vi "Get Largest Decoration Reference.vi"(8 "error in (no error)":errorcluster, 10 "VI reference (calling)":refnum<vi>, 11 "Dialog in":refnum<class "Dialog.lvclass">) -> (0 "error out":errorcluster, 2 "VI reference (dup)":refnum<vi>, 3 "Dialog out":refnum<class "Dialog.lvclass">)   [LabVIEW 2012, in "Dialog.lvlib" / "Dialog.lvclass"]
uses:
  Dialog.lvclass
  Dialog.lvclass/Dialog.ctl
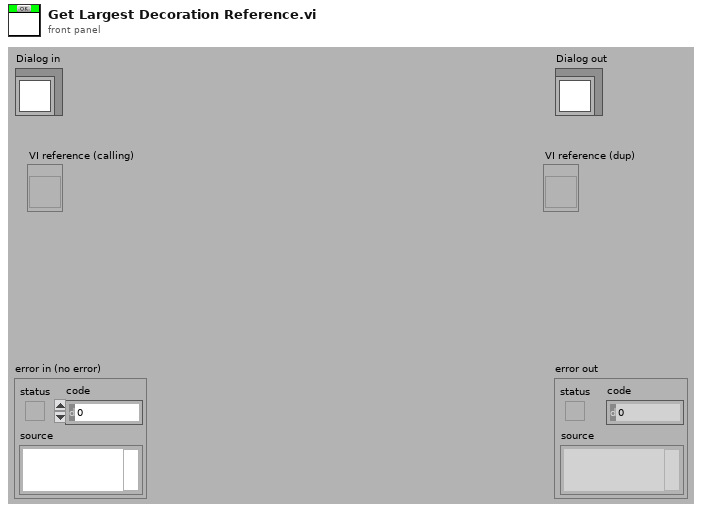
[diagram p1: front panel]
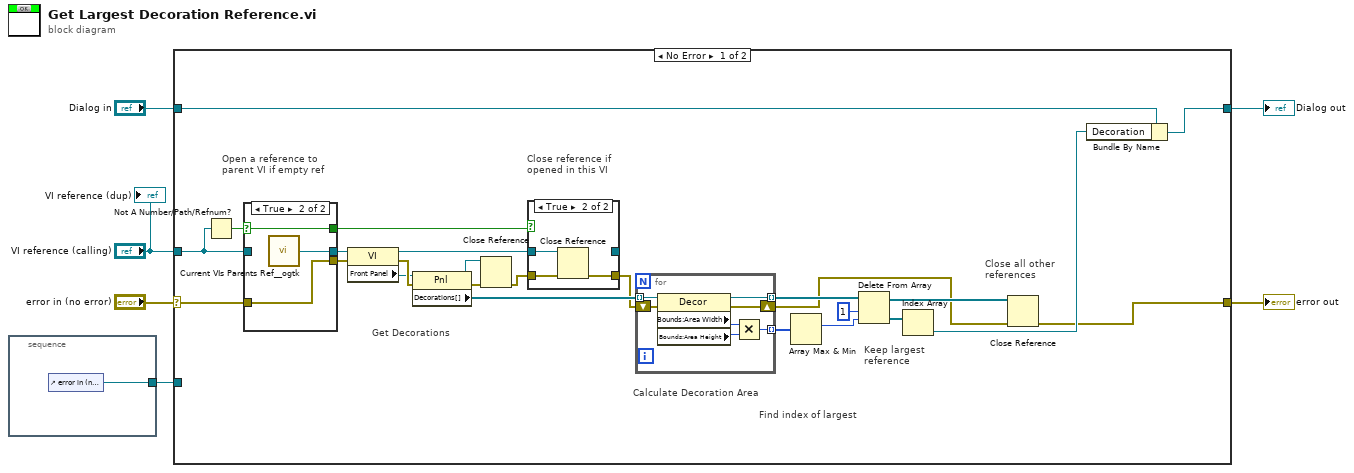
[diagram p0: block diagram]
diagram:
  n1 = stacked-sequence {
    tunnel: [w7] -> w1
    frame #0 {
      n2 = control-ref of="error in (no error)"() -> (w7:refnum<vi>)
    }
  }
  n3 = case shown="No Error" "error in (no error)" {
    selector: "error in (no error)" -> [w25 w52]
    tunnel: [w8 w52] -> w5
    tunnel: [w29 w51] -> w3
    tunnel: "Dialog in" -> [w30 w51]
    tunnel: "VI reference (calling)" -> [w26 _]
    tunnel: w1 -> [_ _]
    frame No Error {
      # "Close all other\nreferences"
      # "Keep largest\nreference"
      # "Find index of largest"
      # "Calculate Decoration Area"
      # "Get Decorations"
      # "Close reference if\nopened in this VI"
      # "Open a reference to\nparent VI if empty ref"
      n4 = Not A Number/Path/Refnum?(number/path/refnum=w26) -> (NaN/Path/Refnum?=w28:bool)
      n5 = case shown="True" w28 {
        selector: w28 -> [w46 w50]
        tunnel: [w46 w50] -> w23
        tunnel: [w47 w49] -> w27
        tunnel: w26 -> [w47 _]
        tunnel: w25 -> [w45 w48]
        tunnel: [w45 w48] -> w24
        frame False {
        }
        frame True {
          n6 = call <userlib>:"Current VIs Parents Ref__ogtk.vi"() -> ("Calling VI's Reference"=w49:refnum<vi>)  [unwired: 2 out]
        }
      }
      n7 = property on="Property Node" class="VI"(reference=w27, error in=w24) -> (reference out=w22:refnum<vi>, error out=w32:errorcluster, "Front Panel"=w31:refnum<vi>)
      n8 = property on="Property Node" class="Pnl"(reference=w31, error in=w32) -> (reference out=w20:refnum<vi>, error out=w21:errorcluster, "Decorations[]"=w18:refnum<vi>[])
      n9 = Close Reference(reference=w20, error in (no error)=w21) -> (error out=w19:errorcluster)
      n10 = case shown="True" w23 {
        tunnel: w22 -> [w40 w44]
        tunnel: [w41 w43] -> w17
        tunnel: w19 -> [w41 w42]
        tunnel: [w40 _] -> _
        frame False {
        }
        frame True {
          n11 = Close Reference(reference=w44, error in (no error)=w42) -> (error out=w43:errorcluster)
        }
      }
      n12 = for {
        tunnel: w18 -> [w39] mode=indexing
        tunnel: [w38] -> w16 mode=indexing
        shift-right: [w36] -> w9
        shift-left: w17 -> [w37]
        tunnel: [w35] -> w15 mode=indexing
        n13 = property class="Decor"(reference=w39, error in=w37) -> (reference out=w35:refnum<vi>, error out=w36:errorcluster, "Bounds:Area Width"=w33:u32, "Bounds:Area Height"=w34:u32)
        n14 = Multiply(x=w33, y=w34) -> (x*y=w38:u32)
      }
      n15 = Array Max & Min(array=w16) -> (max index (indices)=w13:i32)  [unwired: 3 out]
      n16 = Delete From Array(array=w15, length=1, index=w13) -> (deleted portion=w12:refnum<vi>[], array with subset deleted=w10:refnum<vi>[])
      n17 = Index Array(array=w12) -> (element=w11:refnum<vi>)  [unwired: 1 in]
      n18 = Close Reference(reference=w10, error in (no error)=w9) -> (error out=w8:errorcluster)
      n19 = Bundle By Name(cluster=w30, "Decoration"=w11) -> (w29:refnum<class "Dialog.lvclass">)
    }
    frame Error {
    }
  }
  "error out" <- w5
  "Dialog out" <- w3
  "VI reference (dup)" <- "VI reference (calling)"
